vi "ESPI 1.5 modded.vi"() -> ()   [LabVIEW 2013]
uses:
  Instance          21 23Saved   ESPI 1.5 modded .vi
  Instance          20 23Saved   ESPI 1.5 modded .vi
  <vilib>/vision/NI_Vision_Development_Module.lvlib
panel:
  out "Selected Path":path
  in  "Save AVI":bool
  in  "Show ESPI 2":bool=TRUE
  in  "Save Frame":bool
  in  "Number of frames to average\n< 31":i32=30
  in  "Multiplier":dbl=1.0
  in  "Image Type":T1(ring)
  in  "BY FRAME":bool
  in  "Average":bool
  in  "NUMBER OF FRAMES":i32=30
  in  "Palette":T2(ring)
  in  "milliseconds to wait":u32
  in  "Low Pass Filter":bool
  in  "Constant":sgl=42.0 format="%.2f"
  in  "stop":bool
  # "Low Pass Filter"
  # "iMAGE SUBTRACT"
  # "OUTPUT CONTROLS"
  # "Movie"
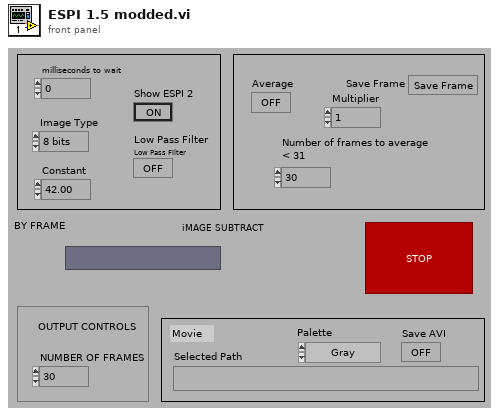
[diagram p1: front panel]
types:
  T1 = enum32{"8 bits", "16 bits", "Float", "Complex", "RGB Chunky", "Compressed"}
  T2 = enum32{"Gray", "Binary", "Gradient", "Rainbow", "Temperature"}
  T3 = cluster{"X Size":i32, "Y Size":i32, "% Tolerance":i32}
  T4 = typedef "IMAQ Image.ctl" = refnum<image>
  T5 = typedef "AviRefnum.ctl" = refnum<k1>
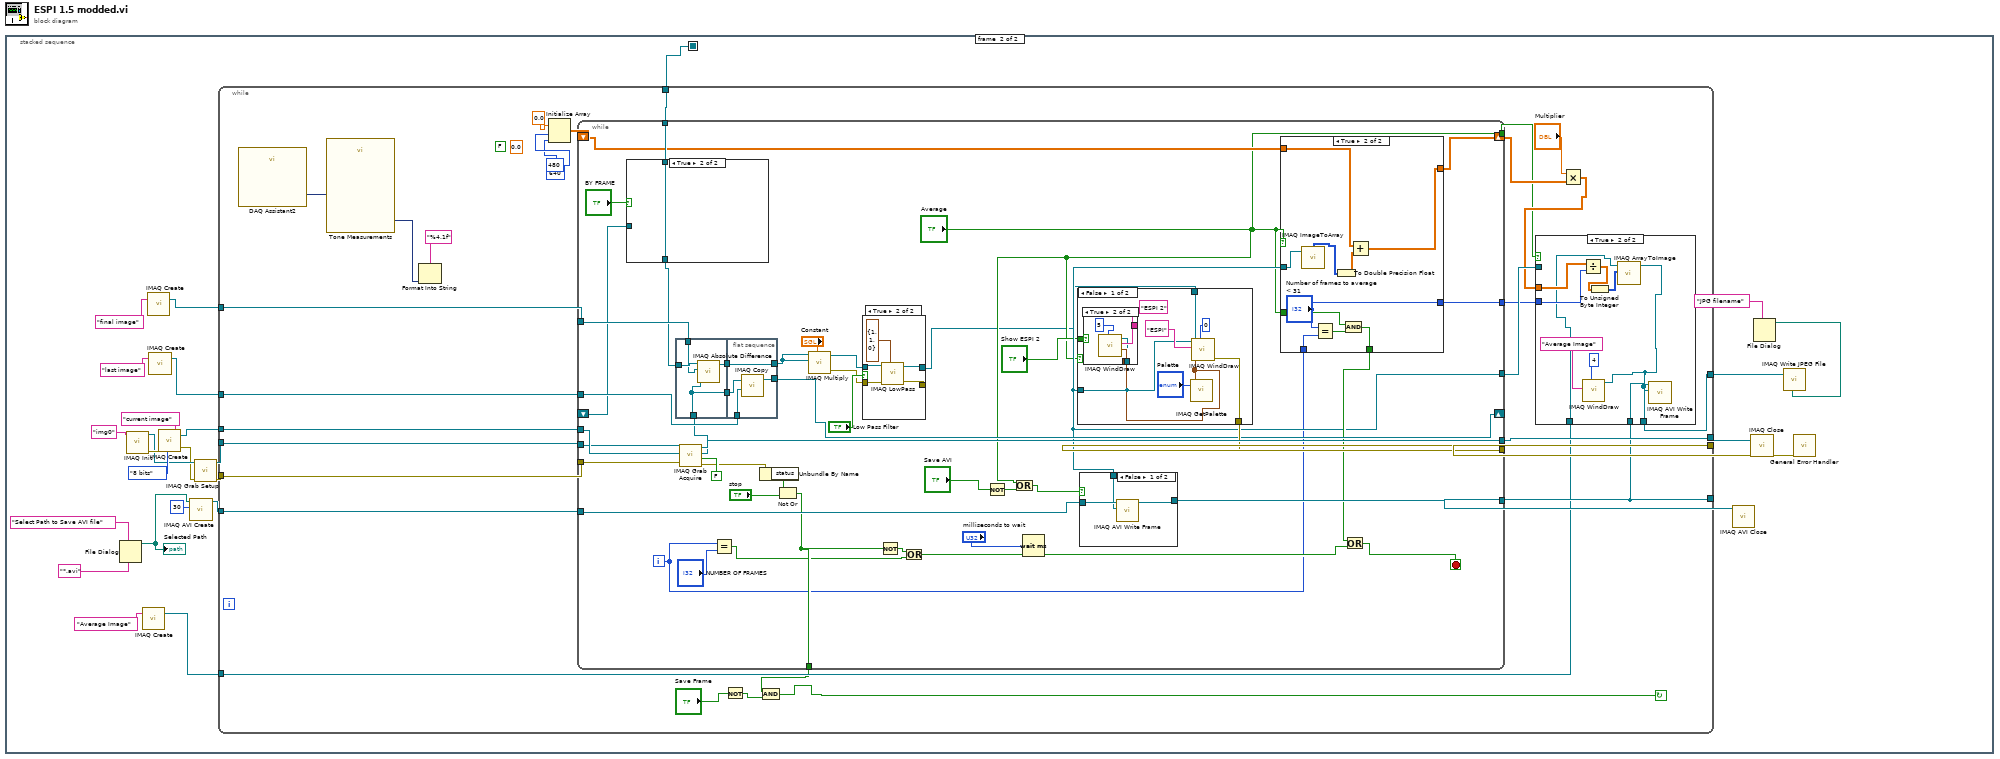
[diagram p0: block diagram]
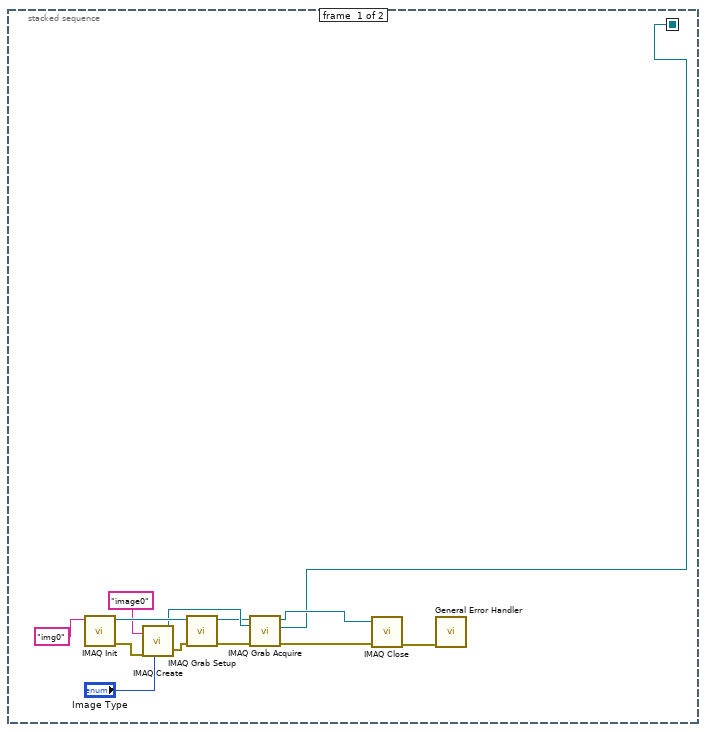
[diagram p2: hidden frame]
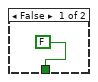
[diagram p8: hidden frame]
diagram:
  n1 = stacked-sequence {
    seq-local: [w1 _] -> [_ w22]
    frame #0 {
      n2 = call <vilib>:"IMAQ Init.vi"("Interface Name"="img0") -> ("error out"=w7:errorcluster, "IMAQ Session Out"=w11:refnum<k11>)  [unwired: 9 in]
      n3 = call "IMAQ Create"("Image Name"="image0", "Image Type"="Image Type", "error in (no error)"=w7) -> ("New Image"=w10:T4, "error out"=w12:errorcluster)  [unwired: 2 in]
      n4 = call <vilib>:"IMAQ Grab Setup.vi"("error in (no error)"=w12, "IMAQ Session In"=w11) -> ("error out"=w8:errorcluster, "IMAQ Session Out"=w9:refnum<k11>)  [unwired: 8 in]
      n5 = call <vilib>:"IMAQ Grab Acquire.vi"("error in (no error)"=w8, "Image In"=w10, "IMAQ Session In"=w9) -> ("error out"=w2:errorcluster, "Image Out"=w1:T4, "IMAQ Session Out"=w4:refnum<k11>)  [unwired: 5 in, 1 out]
      n6 = call <vilib>:"IMAQ Close.vi"("error in (no error)"=w2, "IMAQ Session In"=w4) -> ("error out"=w13:errorcluster)  [unwired: 9 in]
      n7 = call <vilib>:"General Error Handler.vi"("error in (no error)"=w13) -> ()  [unwired: 10 in, 5 out]
    }
    frame #1 {
      n8 = File Dialog(6:"*.avi" ("pattern"), 7:"Select Path to Save AVI file" ("prompt")) -> (3:w15:path)  [unwired: 5 in, 3 out]
      "Selected Path" <- w15
      n9 = call <vilib>:"IMAQ Init.vi"("Interface Name"="img0" ("Current image")) -> ("error out"=w36:errorcluster, "IMAQ Session Out"=w34:refnum<k11>)  [unwired: 9 in]
      n10 = call "IMAQ Create"("Image Name"="Average Image" ("final image")) -> ("New Image"=w19:T4)  [unwired: 4 in, 1 out]
      n11 = call "IMAQ Create"("Image Name"="final image" ("final image")) -> ("New Image"=w26:T4)  [unwired: 4 in, 1 out]
      n12 = call "IMAQ Create"("Image Name"="last image" ("Last image")) -> ("New Image"=w31:T4)  [unwired: 4 in, 1 out]
      n13 = call "IMAQ Create"("Image Name"="current image", "Image Type"=T1."8 bits" ("Image Type 2"), "error in (no error)"=w36) -> ("New Image"=w35:T4, "error out"=w33:errorcluster)  [unwired: 2 in]
      n14 = call "IMAQ AVI Create"("Frames Per Second"=u32 30, "AVI Path"=w15) -> ("Avi Refnum"=w25:T5)  [unwired: 8 in, 1 out]
      n15 = call <vilib>:"IMAQ Grab Setup.vi"("error in (no error)"=w33, "IMAQ Session In"=w34) -> ("error out"=w30:errorcluster, "IMAQ Session Out"=w28:refnum<k11>)  [unwired: 8 in]
      n16 = while {
        tunnel: [w70] -> w40
        tunnel: w35 -> [w69]
        tunnel: w31 -> [w68]
        tunnel: w30 -> [w67]
        tunnel: [w66] -> w29
        tunnel: w28 -> [w65]
        tunnel: w26 -> [w64]
        tunnel: w25 -> [w63]
        tunnel: [w42] -> w24
        tunnel: w22 -> [w61]
        tunnel: [w58] -> w21
        tunnel: w19 -> [w57]
        stop <- w49 continue-if-true
        (unwired) 0.0 ("offset")
        (unwired) FALSE ("reset signal")
        n17 = call "DAQ Assistant2"() -> ("data"=w44:dynamicdata)  [unwired: 9 in, 2 out]
        n18 = call "Tone Measurements"("Signals"=w44) -> ("Frequency"=w45:dynamicdata)  [unwired: 8 in, 2 out]
        n19 = Format Into String(format string="%4.1f", w45) -> ()  [unwired: 2 in, 2 out]
        n20 = Initialize Array(0.0 ("element"), 480 ("dimension size"), 640 ("dimension size")) -> (w53:dbl[][])
        n21 = while {
          tunnel: w68 -> [w106]
          tunnel: w69 -> [w124]
          tunnel: [w125] -> w70
          tunnel: w67 -> [w114]
          tunnel: [w113] -> w66
          tunnel: w65 -> [w112]
          shift-right: [w107] -> _
          shift-left: _ -> [w94]
          tunnel: w64 -> [w111]
          tunnel: w63 -> [w104]
          tunnel: [w103] -> w42
          tunnel: [w102] -> w48
          tunnel: ["Average"] -> w43
          tunnel: w61 -> [w92]
          tunnel: [w90] -> w60
          shift-right: [w91] -> w51
          shift-left: w53 -> [w89]
          tunnel: [w87] -> w59
          i -> [w88]
          stop <- w97 stop-if-true
          n22 = case shown="True" "BY FRAME" {
            tunnel: w94 -> [w144 _]
            tunnel: [w144 w145] -> w93
            tunnel: w92 -> [_ w145]
            frame False {
            }
            frame True {
            }
          }
          n23 = flat-sequence {
            tunnel: w93 -> [w160]
            tunnel: w111 -> [w159]
            tunnel: w105 -> [w157]
            tunnel: [w158] -> w109
            tunnel: [w157] -> w108
            tunnel: [w164] -> w110
            tunnel: w109 -> [w164]
            tunnel: w108 -> [w163]
            tunnel: [w162] -> w107
            tunnel: w106 -> [w161]
            frame #0 {
              n24 = call "IMAQ Absolute Difference"("Image Src A"=w160, "Image Dst"=w159, "Image Src B"=w157) -> ("Image Dst Out"=w158:T4)  [unwired: 4 in, 1 out]
            }
            frame #1 {
              n25 = call "IMAQ Copy"("Image Dst"=w161, "Image Src"=w163) -> ("Image Dst Out"=w162:T4)  [unwired: 4 in, 1 out]
            }
          }
          n26 = call <vilib>:"IMAQ Grab Acquire.vi"("error in (no error)"=w114, "Immediate?"=FALSE ("Immediate ?"), "Image In"=w124, "IMAQ Session In"=w112) -> ("error out"=w116:errorcluster, "Image Out"=w105:T4, "IMAQ Session Out"=w125:refnum<k11>)  [unwired: 4 in, 1 out]
          n27 = Equal?(x=w88, y="NUMBER OF FRAMES") -> (x = y?=w99:bool)
          n28 = Unbundle By Name(w116) -> ("status"=w123:bool)
          n29 = Not Or(1:"stop", 2:w123) -> (0:w102:bool)
          n30 = call "IMAQ Multiply"("Image Src A"=w110, "Constant"="Constant", "Image Dst"=w110) -> ("Image Dst Out"=w118:T4, "error out"=w117:errorcluster)  [unwired: 4 in]
          n31 = case shown="True" "Low Pass Filter" {
            tunnel: [w166 w170] -> _
            tunnel: w118 -> [w165 w168]
            tunnel: [w165 w169] -> w81
            tunnel: w117 -> [w166 w171]
            frame False {
            }
            frame True {
              n32 = call "IMAQ LowPass"("Image Src"=w168, "Size & Tolerance"=T3 {"X Size"=1, "Y Size"=1, "% Tolerance"=0}, "error in (no error)"=w171) -> ("Image Dst Out"=w169:T4, "error out"=w170:errorcluster)  [unwired: 4 in]
            }
          }
          n33 = Not(x=w102) -> (.not. x?=w101:bool)
          n34 = Or(x=w101, y=w99) -> (x .or. y?=w98:bool)
          n35 = Not(x="Save AVI") -> (.not. x?=w83:bool)
          n36 = Or(x="Average", y=w83) -> (x .or. y?=w84:bool)
          n37 = Wait (ms)(milliseconds to wait="milliseconds to wait") -> ()  [unwired: 1 out]
          n38 = case shown="False" "Average" {
            tunnel: [w132 _] -> w113
            tunnel: w81 -> [w136 w143]
            tunnel: [w131 w143] -> w90
            tunnel: "Show ESPI 2" -> [w130 _]
            frame False {
              n39 = call "IMAQ GetPalette"("Palette Number (gray)"="Palette") -> ("Color Palette"=w133:cluster{"Red":u8, "Green":u8, "Blue":u8}[])  [unwired: 4 in, 1 out]
              n40 = call "IMAQ WindDraw"("Window Number (0...15)"=0, "Color Palette"=w133, "Title"="ESPI", "Image"=w136) -> ("error out"=w132:errorcluster, "Image Out (duplicate)"=w131:T4)  [unwired: 6 in]
              n41 = case shown="True" w130 {
                tunnel: "ESPI 2" ("Title") -> [_ w142]
                tunnel: w133 -> [_ w141]
                tunnel: w131 -> [_ w140]
                frame False {
                }
                frame True {
                  n42 = call "IMAQ WindDraw"("Window Number (0...15)"=5, "Color Palette"=w141, "Title"=w142, "Image"=w140) -> ()  [unwired: 6 in, 2 out]
                }
              }
            }
            frame True {
            }
          }
          n43 = case shown="False" w84 {
            tunnel: w104 -> [w128 w129]
            tunnel: [w127 w129] -> w103
            tunnel: w90 -> [w126 _]
            frame False {
              n44 = call "IMAQ AVI Write Frame"("Image"=w126, "Avi Refnum"=w128) -> ("Avi Refnum (duplicate)"=w127:T5)  [unwired: 8 in, 1 out]
            }
            frame True {
            }
          }
          n45 = case shown="True" "Average" {
            tunnel: w90 -> [_ w156]
            tunnel: [_ w152] -> w91
            tunnel: [FALSE w155] -> w96
            tunnel: "Average" -> [_ w153]
            tunnel: w89 -> [_ w151]
            tunnel: w88 -> [_ w150]
            tunnel: [_ "Number of frames to average\n< 31"] -> w87
            frame False {
            }
            frame True {
              n46 = call "IMAQ ImageToArray"("Image"=w156) -> ("Image Pixels (U8)"=w148:u8[][])  [unwired: 3 in, 4 out]
              n47 = Equal?(x="Number of frames to average\n< 31", y=w150) -> (x = y?=w154:bool)
              n48 = To Double Precision Float(number=w148) -> (double precision float=w147:dbl[][])
              n49 = And(x=w153, y=w154) -> (x .and. y?=w155:bool)
              n50 = Add(x=w151, y=w147) -> (x+y=w152:dbl[][])
            }
          }
          n51 = Or(x=w96, y=w98) -> (x .or. y?=w97:bool)
        }
        n52 = Not(x="Save Frame") -> (.not. x?=w46:bool)
        n53 = And(x=w48, y=w46) -> (x .and. y?=w49:bool)
        n54 = Multiply(x="Multiplier", y=w51) -> (x*y=w50:dbl[][])
        n55 = case shown="True" w43 {
          tunnel: w50 -> [_ w78]
          tunnel: [w71 w72] -> w58
          tunnel: w60 -> [w71 _]
          tunnel: w59 -> [_ w77]
          tunnel: w57 -> [_ w74]
          tunnel: w42 -> [_ w73]
          frame False {
          }
          frame True {
            n56 = Divide(x=w78, y=w77) -> (x/y=w80:dbl[][])
            n57 = To Unsigned Byte Integer(number=w80) -> (unsigned 8bit integer=w79:u8[][])
            n58 = call "IMAQ ArrayToImage"("Image Pixels (U8)"=w79, "Image"=w74) -> ("Image Out"=w72:T4)  [unwired: 8 in, 1 out]
            n59 = call "IMAQ WindDraw"("Window Number (0...15)"=4, "Title"="Average Image", "Image"=w72) -> ()  [unwired: 7 in, 2 out]
            n60 = call "IMAQ AVI Write Frame"("Image"=w72, "Avi Refnum"=w73) -> ()  [unwired: 8 in, 2 out]
          }
        }
      }
      n61 = call "IMAQ AVI Close"("Avi Refnum"=w24) -> ()  [unwired: 10 in, 1 out]
      n62 = call <vilib>:"IMAQ Close.vi"("error in (no error)"=w29, "IMAQ Session In"=w40) -> ("error out"=w41:errorcluster)  [unwired: 9 in]
      n63 = File Dialog(7:"JPG filename" ("prompt")) -> (3:w18:path)  [unwired: 6 in, 3 out]
      n64 = call "IMAQ Write JPEG File"("File Path"=w18, "Image"=w21) -> ()  [unwired: 6 in, 1 out]
      n65 = call <vilib>:"General Error Handler.vi"("error in (no error)"=w41) -> ()  [unwired: 10 in, 5 out]
    }
  }
